vi "RP1210 Get Hardware Status.vi"(8 "error in (no error)":errorcluster, 9 "nBlockOnRequest":i16, 10 "nInfoSize":i16=18, 11 "nClientID":i16) -> (0 "error out":errorcluster, 2 "function return":i16, 3 "fpchClientInfo":u8[](array[numeric]))   [LabVIEW 2020, in "cansub_rp1210.lvlib"]
doc: "short __stdcall RP1210_GetHardwareStatus(short nClientID, unsigned char fpchClientInfo[], short nInfoSize,\n short nBlockOnRequest);"
uses:
  cansub_rp1210.lvlib
  cansub_lv64.dll
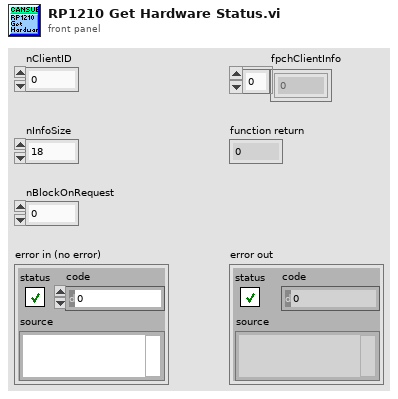
[diagram p1: front panel]
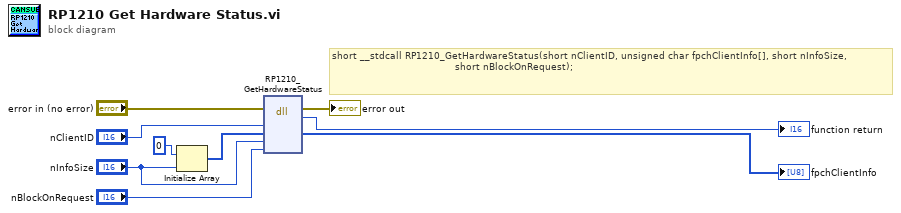
[diagram p0: block diagram]
diagram:
  # "short __stdcall RP1210_GetHardwareStatus(short nClientID, unsigned char fpchClientInfo[], short nInfoSize,\n                                         short nBlockOnRequest);"
  n1 = Initialize Array(u8 0 ("element"), "nInfoSize") -> (w7:u8[])
  n2 = dll-call lib="C:/cansub-lv/library/cansub_lv*.*" fn="RP1210_GetHardwareStatus"(error in="error in (no error)", "nClientID"="nClientID", "fpchClientInfo"=w7, "nInfoSize"="nInfoSize", "nBlockOnRequest"="nBlockOnRequest") -> (error out=→"error out":errorcluster, "return type"=→"function return":i16, "fpchClientInfo"=→"fpchClientInfo":u8[])  [unwired: 5 in, 1 out]
